vi "Installer Pre-Uninstall Action.vi"() -> ()   [LabVIEW 2015]
panel:
  out "error out":errorcluster
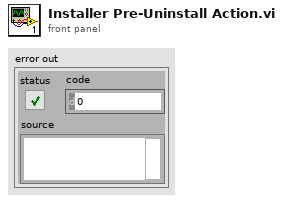
[diagram p1: front panel]
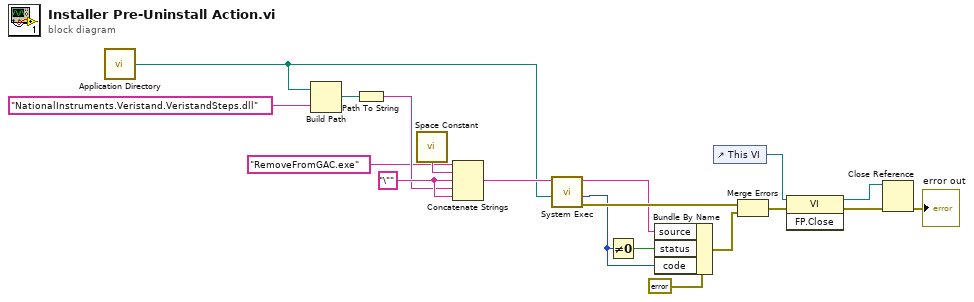
[diagram p0: block diagram]
diagram:
  w19 = "\"" ("string")
  n1 = call <vilib>:"Application Directory.vi"() -> ("Application Directory"=w12:path)
  n2 = Build Path(base path=w12, name or relative path="NationalInstruments.Veristand.VeristandSteps.dll" ("command line")) -> (appended path=w17:path)
  n3 = Path To String(path=w17) -> (string=w15:string)
  n4 = call <vilib>:"Space Constant.vi"() -> ("String"=w18:string)
  n5 = Concatenate Strings("RemoveFromGAC.exe" ("string"), w18, w19, w15, w19) -> (w13:string)
  n6 = call <vilib>:"System Exec.vi"("working directory"=w12, "command line"=w13) -> ("error out"=w6:errorcluster, "return code"=w3:i32, "standard output"=w2:string)  [unwired: 6 in, 1 out]
  n7 = Not Equal To 0?(x=w3) -> (x != 0?=w4:bool)
  n8 = Bundle By Name(cluster=errorcluster {"status"=FALSE, "code"=0, "source"=""} ("error in"), "source"=w2, "status"=w4, "code"=w3) -> (w1:errorcluster)
  n9 = control-ref of="This VI"() -> (w11:refnum<vi>)
  n10 = Merge Errors(w6, w1) -> (w7:errorcluster)
  n11 = invoke class="VI" method="FP.Close"(reference=w11, error in=w7) -> (reference out=w9:refnum<vi>, error out=w10:errorcluster)  [unwired: 1 in, 1 out]
  n12 = Close Reference(reference=w9, error in (no error)=w10) -> (error out=→"error out":errorcluster)
